vi "Heater compressor control.vi"(0 "VISA resource name":refnum<visa-resource-name>, 5 "UCP":bool, 7 "Heater on":bool, 9 "LCP":bool, 11 "error in":errorcluster) -> (4 "VISA resource name out":refnum<visa-resource-name>, 15 "error out":errorcluster)   [LabVIEW 2026]
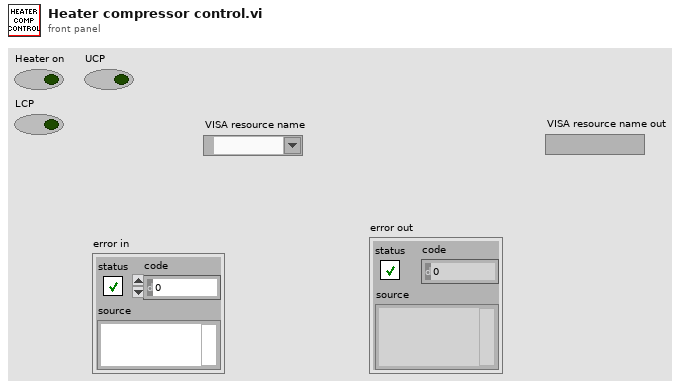
[diagram p1: front panel]
types:
  T1 = cluster{"Mode":enum16{"RTU", "ASCII"}, "Slave Address":u8}
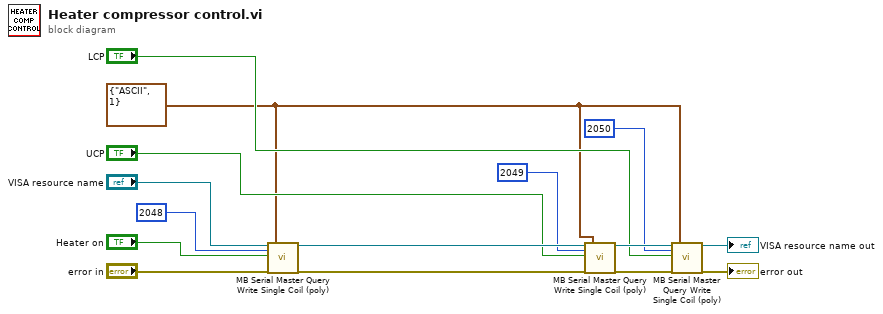
[diagram p0: block diagram]
diagram:
  w3 = T1 {"Mode"=enum."ASCII", "Slave Address"=1} ("Serial Parameters")
  n1 = call <userlib>:"MB Serial Master Query Write Single Coil (poly).vi"("VISA resource name"="VISA resource name", "Address"=u16 2048 ("address"), "Coil"="Heater on", "error in"="error in", "Serial Parameters"=w3) -> ("VISA resource name out"=w14:refnum<visa-resource-name>, "error out"=w13:errorcluster)  [unwired: 12 in, 1 out]
  n2 = call <userlib>:"MB Serial Master Query Write Single Coil (poly).vi"("VISA resource name"=w14, "Address"=u16 2049 ("address"), "Coil"="UCP", "error in"=w13, "Serial Parameters"=w3) -> ("VISA resource name out"=w12:refnum<visa-resource-name>, "error out"=w11:errorcluster)  [unwired: 12 in, 1 out]
  n3 = call <userlib>:"MB Serial Master Query Write Single Coil (poly).vi"("VISA resource name"=w12, "Address"=u16 2050 ("address"), "Coil"="LCP", "error in"=w11, "Serial Parameters"=w3) -> ("VISA resource name out"=→"VISA resource name out":refnum<visa-resource-name>, "error out"=→"error out":errorcluster)  [unwired: 12 in, 1 out]
